vi "vi_get_callees.vi"(10 "VI":refnum<class "HierarchyNode.lvclass">, 11 "Hierarchy":refnum<class "HierarchyGraph.lvclass">) -> (1 "Callees":refnum<class "HierarchyNode.lvclass">[](array[class]), 2 "VI not found?":bool)   [LabVIEW 2020, in "vi-hierarchy.lvlib" / "HierarchyGraph.lvclass"]
uses:
  HierarchyGraph.lvclass
  C:/Projects/labview-project-load-tools/source/submodules/graph-api-labview/source/api/DiGraph/DiGraph.lvclass
  VINode/HierarchyNode.lvclass
  C:/Projects/labview-project-load-tools/source/submodules/graph-api-labview/source/api/Node/Node.lvclass
  api/DiGraph/DiGraph.lvclass
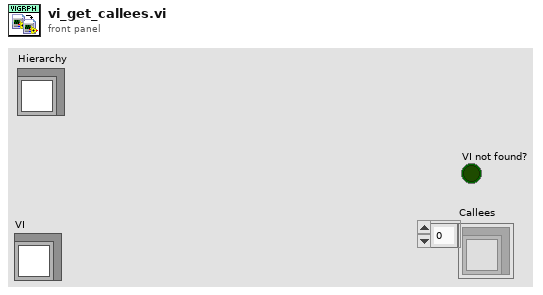
[diagram p1: front panel]
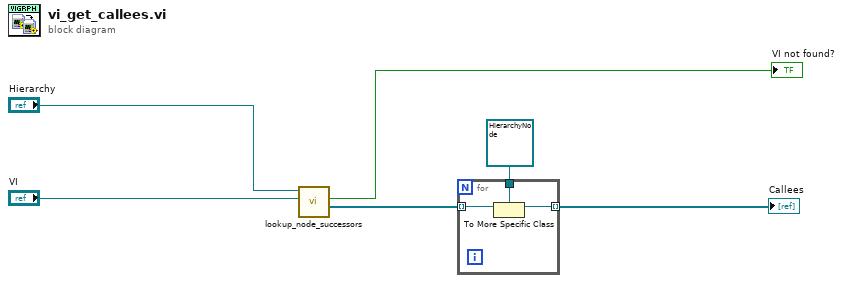
[diagram p0: block diagram]
diagram:
  n1 = call "lookup_node_successors.vi"("node"="VI", "digraph"="Hierarchy") -> ("successors"=w2:refnum<class "Node.lvclass">[], "node not found?"=→"VI not found?":bool)  [unwired: 8 in]
  n2 = for {
    tunnel: w2 -> [w9] mode=indexing
    tunnel: [w8] -> w4 mode=indexing
    tunnel: refnum<class "HierarchyNode.lvclass"> refnum ("VINode") -> [w7]
    n3 = To More Specific Class(target class=w7, reference=w9) -> (specific class reference=w8:refnum<class "HierarchyNode.lvclass">)  [unwired: 1 in, 1 out]
  }
  "Callees" <- w4
